vi "Example Binary.vi"() -> ()   [LabVIEW 2020]
uses:
  <vilib>/Utility/sysdir.llb/System Directory Type.ctl
  Sources/_Helpers/Tiff Page Details.ctl
  Sources/TIFF Writer/TIFF Writer.lvclass
  Sources/LV Tiff.lvlib
  Sources/TIFF Reader/TIFF Reader.lvclass
panel:
  out "Read":u8[][](graph)
  out "Write":u8[][](graph)
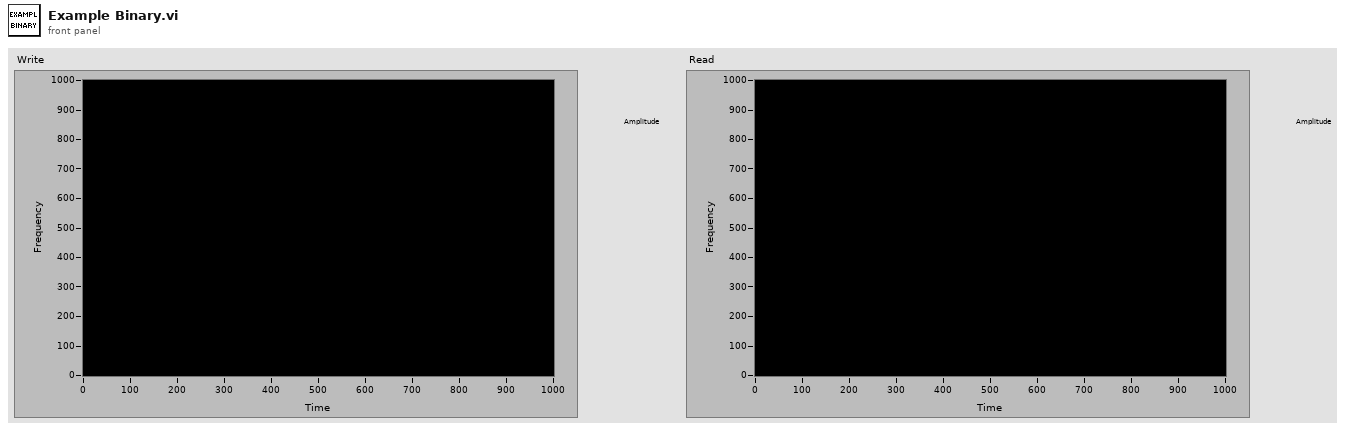
[diagram p1: front panel]
types:
  T1 = typedef "LV Tiff.lvlib/Tiff Page Details.ctl" = cluster{"ImageDescription":string, "XResolution":dbl, "YResolution":dbl, "ResolutionUnit":enum16{"None", "Inch", "Centimeter"}, "PhotometricInterpretation":u16, "Compression":enum16{"None", "Deflate", "JPEG"}, "PageName":string, "DocumentName":string}
  T2 = enum16{"open", "replace", "create", "open or create", "replace or create", "replace or create with confirmation"}
  T3 = typedef "System Directory Type.ctl" = i32
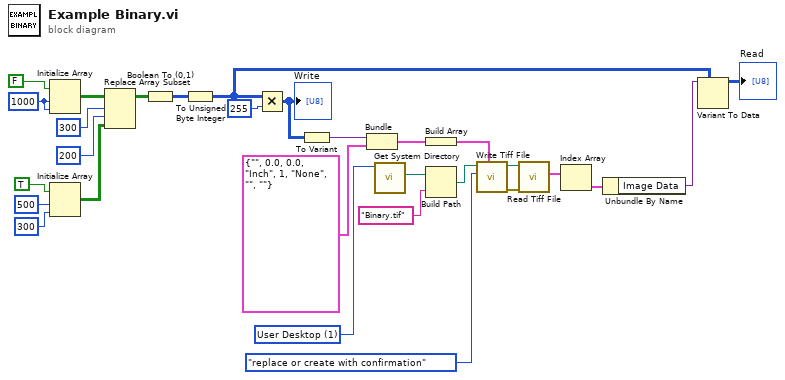
[diagram p0: block diagram]
diagram:
  w29 = T3 1 items=["User Home"=0, "User Desktop"=1, "User Documents"=2, "User Application Data"=3, "User Preferences"=4, "User Temporary"=5, "Public Documents"=6, "Public Application Data"=7, "Public Preferences"=8, "Public Cache"=13, "System Core Libraries"=9, "System Installed Libraries"=10, "Application Files"=11, "Boot Volume Root"=12] ("system directory type")
  w17 = 1000
  n1 = Initialize Array(FALSE, w17, w17) -> (w18:bool[][])
  n2 = Initialize Array(TRUE ("element"), 500 ("dimension size"), 300 ("dimension size")) -> (w12:bool[][])
  n3 = Replace Array Subset(array=w18, new element=w12, index (row)=300, index (col)=200 ("disabled index (col)")) -> (w4:bool[][])
  n4 = Boolean To (0,1)(Boolean=w4) -> (0, 1=w20:i16[][])
  n5 = To Unsigned Byte Integer(number=w20) -> (unsigned 8bit integer=w3:u8[][])
  n6 = Multiply(x=w3, y=u8 255) -> (x*y=w1:u8[][])
  "Write" <- w1
  n7 = To Variant(anything=w1) -> (Variant=w24:variant)
  n8 = Bundle("Variant"=w24, "Details"=T1 {"ImageDescription"="", "XResolution"=0.0, "YResolution"=0.0, "ResolutionUnit"=enum."Inch", "PhotometricInterpretation"=1, "Compression"=enum."None", "PageName"="", "DocumentName"=""}) -> (w22:cluster{"Variant":variant, "Details":T1})  [unwired: 1 in]
  n9 = call <vilib>:"Get System Directory.vi"("system directory type"=w29) -> ("system directory"=w28:path)  [unwired: 10 in]
  n10 = Build Array(w22) -> (w21:cluster{"Variant":variant, "Details":T1}[])
  n11 = Build Path(base path=w28, name or relative path="Binary.tif") -> (appended path=w26:path)
  n12 = call "Write Tiff File.vi"("Pages"=w21, "operation (replace)"=T2."replace or create with confirmation", "Path"=w26) -> ("error out"=w8:errorcluster, "path"=w9:path)  [unwired: 7 in]
  n13 = call "Read Tiff File.vi"("error in (no error)"=w8, "Path"=w9) -> ("Pages"=w7:cluster{"Image Data":variant, "Details":T1}[])  [unwired: 6 in, 3 out]
  n14 = Index Array(array=w7) -> (element=w6:cluster{"Image Data":variant, "Details":T1})  [unwired: 1 in]
  n15 = Unbundle By Name(w6) -> ("Image Data"=w5:variant)
  n16 = Variant To Data(type=w3, Variant=w5) -> (data=→"Read":u8[][])  [unwired: 1 in, 1 out]
